vi "子VI-Readx.vi"(0 "会话":u32, 1 "指令":string, 2 "超时":u32, 3 "长度":u32, 4 "数据":dbl[](array[numeric])) -> (5 "描述":string, 6 "返回值":i32)   [LabVIEW 2011]
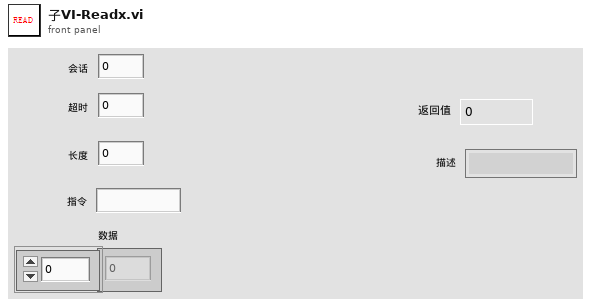
[diagram p1: front panel]
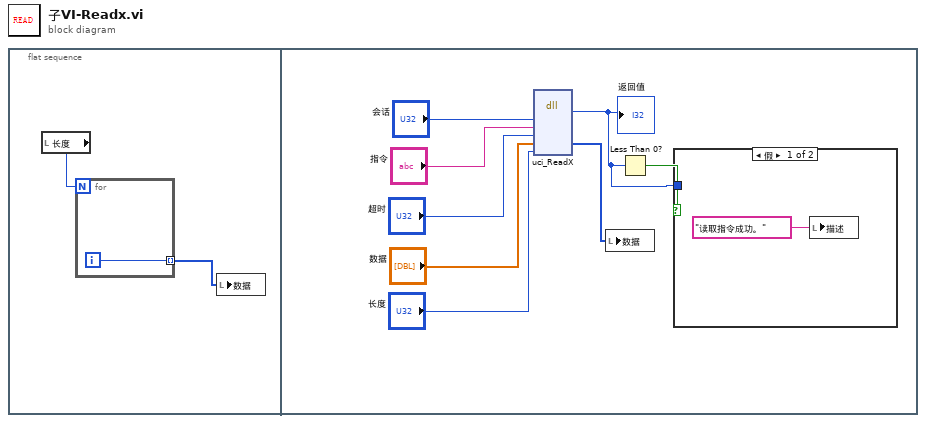
[diagram p0: block diagram]
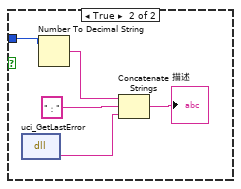
[diagram p2: hidden frame]
diagram:
  n1 = flat-sequence {
    frame #0 {
      n2 = local read "长度"() -> (w2:u32)
      n3 = for {
        N: w2 -> [_]
        tunnel: [w3] -> w1 mode=indexing
        i -> [w3]
      }
      n4 = local write "数据"(w1) -> ()
    }
    frame #1 {
      n5 = dll-call lib="PTH1Eabs E调试程序\nLabView程序UCI示例程序ASCIIuci.dll" fn="uci_ReadX"("session"="会话", "msg"="指令", "timeout"="超时", "data"="数据", "len"="长度") -> ("返回类型"=w4:i32, "data"=w5:u8[])  [unwired: 7 in, 2 out]
      "返回值" <- w4
      n6 = local write "数据"(w5) -> ()
      n7 = Less Than 0?(x=w4) -> (x < 0?=w6:bool)
      n8 = case shown="假" w6 {
        tunnel: w4 -> [_ w13]
        frame False {
          n9 = local write "描述"("读取指令成功。") -> ()
        }
        frame True {
          n10 = dll-call lib="PTH1Eabs E调试程序\nLabView程序UCI示例程序ASCIIuci.dll" fn="uci_GetLastError"() -> ("返回类型"=w15:string)  [unwired: 3 in, 2 out]
          n11 = Number To Decimal String(number=w13) -> (decimal integer string=w17:string)  [unwired: 1 in]
          n12 = Concatenate Strings(w17, "：", w15) -> (→"描述":string)
        }
      }
    }
  }
